vi "Set_Accel_Decel.vi"(8 "error in (no error)":errorcluster, 9 "Decel (ms/krpm)":u16=200, 10 "Accel (ms/krpm)":u16=200, 11 "WEG_SCA06_Modbus in":refnum<class "WEG_SCA06_Modbus.lvclass">) -> (0 "error out":errorcluster, 3 "WEG_SCA06_Modbus out":refnum<class "WEG_SCA06_Modbus.lvclass">)   [LabVIEW 2021, in "WEG_SCA06_Modbus.lvclass"]
uses:
  WEG_SCA06_Modbus.lvclass
  WEG_SCA06_Modbus.lvclass/WEG_SCA06_Modbus.ctl
  Modbus_Master/Modbus_Master.lvclass
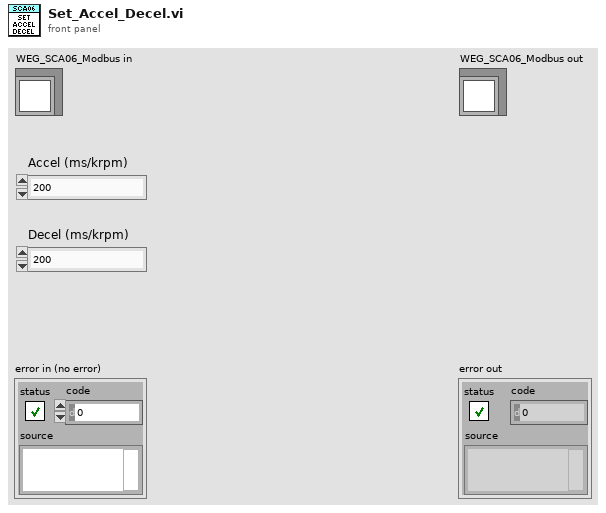
[diagram p1: front panel]
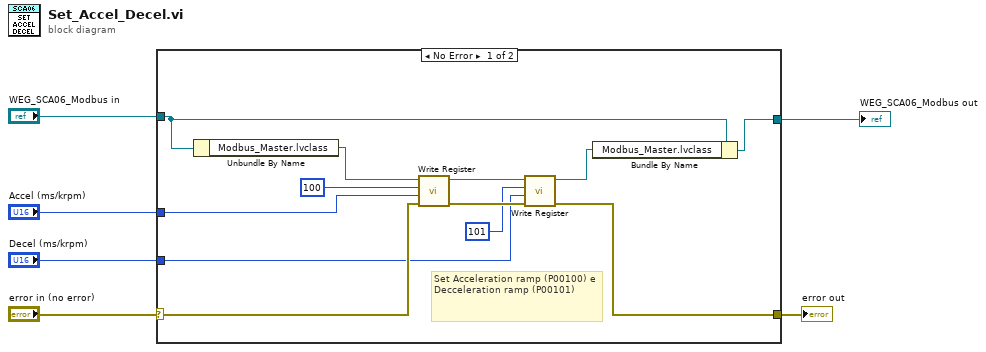
[diagram p0: block diagram]
diagram:
  n1 = case shown="No Error" "error in (no error)" {
    selector: "error in (no error)" -> [w15 w19]
    tunnel: "WEG_SCA06_Modbus in" -> [w18 w20]
    tunnel: [w17 w20] -> w4
    tunnel: [w12 w19] -> w3
    tunnel: "Accel (ms/krpm)" -> [w9 _]
    tunnel: "Decel (ms/krpm)" -> [w7 _]
    frame No Error {
      # "Set Acceleration ramp (P00100) e\nDecceleration ramp (P00101)"
      n2 = Unbundle By Name(w18) -> ("Modbus_Master.lvclass"=w16:refnum<class "Modbus_Master.lvclass">)
      n3 = call "Write Register.vi"("error in (no error)"=w15, "Value"=w9, "Register Address"=u16 100, "Modbus_Master in"=w16) -> ("error out"=w13:errorcluster, "Modbus_Master out"=w14:refnum<class "Modbus_Master.lvclass">)  [unwired: 6 in]
      n4 = call "Write Register.vi"("error in (no error)"=w13, "Value"=w7, "Register Address"=u16 101, "Modbus_Master in"=w14) -> ("error out"=w12:errorcluster, "Modbus_Master out"=w11:refnum<class "Modbus_Master.lvclass">)  [unwired: 6 in]
      n5 = Bundle By Name(cluster=w18, "Modbus_Master.lvclass"=w11) -> (w17:refnum<class "WEG_SCA06_Modbus.lvclass">)
    }
    frame Error {
    }
  }
  "error out" <- w3
  "WEG_SCA06_Modbus out" <- w4
